vi "Execute Command.vi"(7 "Execution Mode (Default: Serialized)":T1, 8 "error in (no error)":errorcluster, 10 "Command":string, 11 "Camera in":refnum<class "Camera.lvclass">) -> (0 "error out":errorcluster, 3 "Camera":refnum<class "Camera.lvclass">)   [LabVIEW 2020, in "Camera.lvclass"]
uses:
  Camera.lvclass
  Execution Mode.ctl
  Camera.lvclass/Camera.ctl
  bin/gindustrialcam_32-1.dll
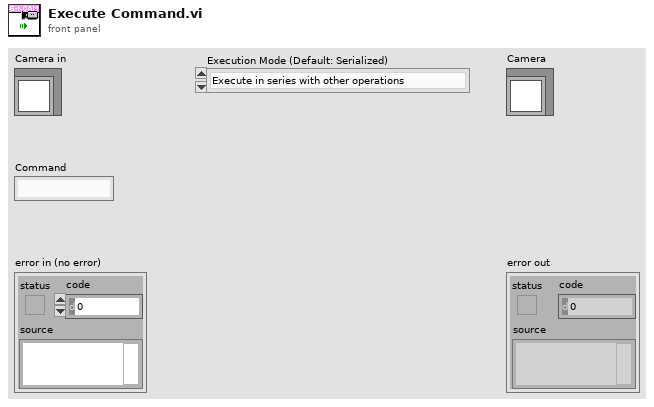
[diagram p1: front panel]
types:
  T1 = typedef "Camera.lvclass/Execution Mode.ctl" = enum16{"Execute in series with other operations", "Execute in parallel with other operations"}
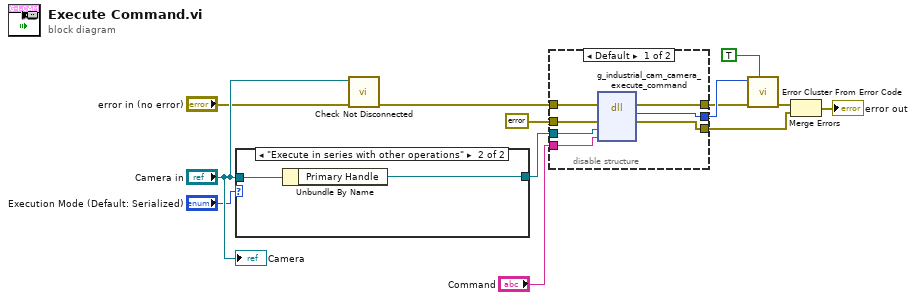
[diagram p0: block diagram]
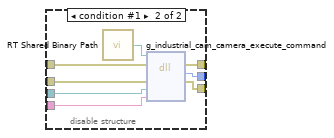
[diagram p2: hidden frame]
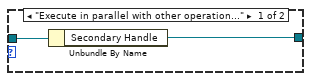
[diagram p3: hidden frame]
diagram:
  n1 = case shown="\"Execute in series with other operations\"" "Execution Mode (Default: Serialized)" {
    tunnel: "Camera in" -> [w15 w17]
    tunnel: [w14 w16] -> w9
    frame "Execute in parallel with other operations" {
      n2 = Unbundle By Name(w15) -> ("Secondary Handle"=w14:refnum<data-value>)
    }
    frame "Execute in series with other operations" {
      n3 = Unbundle By Name(w17) -> ("Primary Handle"=w16:refnum<data-value>)
    }
  }
  n4 = call "Check Not Disconnected.vi"("error in (no error)"="error in (no error)", "Camera in"="Camera in") -> ("error out"=w10:errorcluster)  [unwired: 9 in]
  n5 = disable-structure shown="Default" {
    disable-tunnel: w10 -> [w24 w32]
    disable-tunnel: w9 -> [w23 w31]
    disable-tunnel: errorcluster {"status"=FALSE, "code"=0, "source"=""} ("error constant") -> [w22 w30]
    disable-tunnel: [w21 w29] -> w6
    disable-tunnel: [w20 w28] -> w4
    disable-tunnel: [w19 w27] -> w3
    disable-tunnel: "Command" -> [w18 w26]
    frame condition #0 (active) {
      n6 = dll-call lib="C:/serenial/lib/g-industrial-camera/LabVIEW/g_industrial_cam/bin/gindustrialcam_*-1.*" fn="g_industrial_cam_camera_execute_command"(error in=w24, "err"=w22, "edvr"=w23, "command"=w18) -> (error out=w19:errorcluster, "Mg_Error"=w20:i32, "err"=w21:errorcluster)  [unwired: 4 in, 1 out]
    }
    frame condition #1 {
      n7 = call "RT Shared Binary Path.vi"() -> ("Path"=w25:path)
      n8 = dll-call lib="C:/serenial/lib/g-industrial-camera/LabVIEW/g_industrial_cam/bin/gindustrialcam_*-1.*" fn="g_industrial_cam_camera_execute_command"(path in=w25, error in=w32, "err"=w30, "edvr"=w31, "command"=w26) -> (error out=w27:errorcluster, "Mg_Error"=w28:i32, "err"=w29:errorcluster)  [unwired: 3 in, 1 out]
    }
  }
  n9 = call <vilib>:"Error Cluster From Error Code.vi"("show call chain? (False)"=TRUE, "error in (no error)"=w3, "error code (0)"=w4) -> ("error out"=w5:errorcluster)  [unwired: 6 in]
  n10 = Merge Errors(w5, w6) -> (→"error out":errorcluster)
  "Camera" <- "Camera in"
